vi "Parse String.vi"(8 "error in (no error)":errorcluster, 10 "Input String":string, 11 "ConfigManager.Text in":refnum<class "ConfigManager.Text.lvclass">) -> (0 "error out":errorcluster, 1 "Content":T1[](array[typedef]), 2 "Keys":string[](array[string]), 3 "ConfigManager.Text out":refnum<class "ConfigManager.Text.lvclass">, 5 "Section":string[](array[string]))   [LabVIEW 2013, in "CfgManager.Text.lvlib" / "ConfigManager.Text.lvclass"]
uses:
  ConfigManager.Text.lvclass
  Dictionary Payload -- cluster.ctl
  ConfigManager.Text.lvclass/ConfigManager.Text.ctl
  <vilib>/LabVIEW Open Source Project/Unicity/Delimiter/Delimiter.lvclass
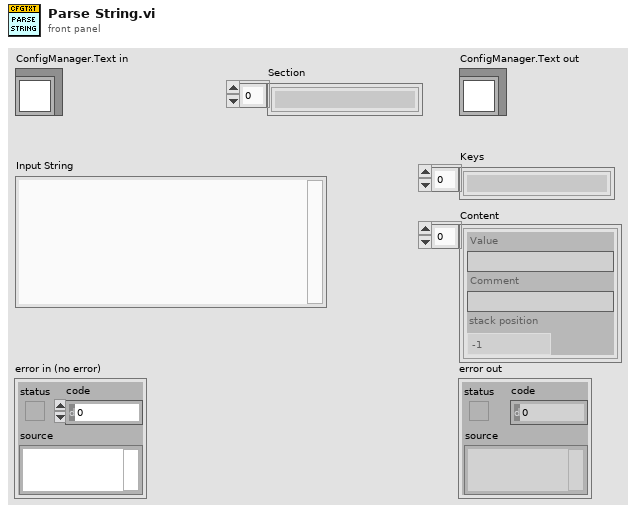
[diagram p1: front panel]
types:
  T1 = typedef "CfgManager.Text.lvlib/ConfigManager.Text.lvclass/Dictionary Payload -- cluster.ctl" = cluster{"Value":string, "Comment":string, "stack position":i32}
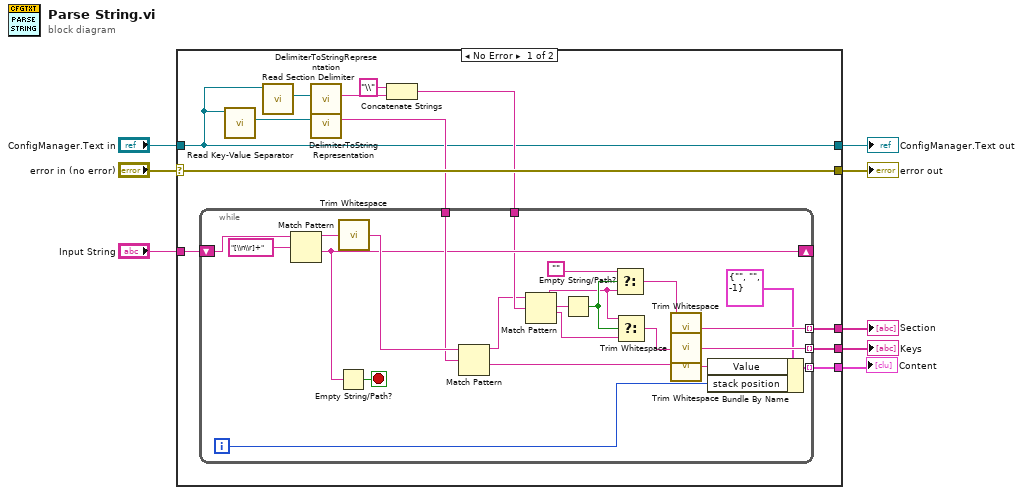
[diagram p0: block diagram]
diagram:
  n1 = case shown="No Error" "error in (no error)" {
    selector: "error in (no error)" -> [w20 w45]
    tunnel: [w20 w45] -> w7
    tunnel: [w10 w44] -> w5
    tunnel: "ConfigManager.Text in" -> [w10 w44]
    tunnel: "Input String" -> [w9 _]
    tunnel: [w19 _] -> w3
    tunnel: [w18 _] -> w1
    tunnel: [w16 _] -> w2
    frame No Error {
      n2 = call "Read Key-Value Separator.vi"("ConfigManager.Text in"=w10) -> ("Key Value Separator"=w11:refnum<class "Delimiter.lvclass">)  [unwired: 9 in, 1 out]
      n3 = call "Read Section Delimiter.vi"("ConfigManager.Text in"=w10) -> ("Section Delimiter"=w12:refnum<class "Delimiter.lvclass">)  [unwired: 9 in, 1 out]
      n4 = call <vilib>:"DelimiterToStringRepresentation.vi"("Delimiter"=w12) -> ("String representation"=w15:string)  [unwired: 10 in]
      n5 = call <vilib>:"DelimiterToStringRepresentation.vi"("Delimiter"=w11) -> ("String representation"=w17:string)  [unwired: 10 in]
      n6 = Concatenate Strings("\\" ("string"), w15) -> (w13:string)
      n7 = while {
        shift-right: [w35] -> _
        shift-left: w9 -> [w42]
        tunnel: [w38] -> w19 mode=indexing
        tunnel: w17 -> [w36]
        tunnel: [w22] -> w18 mode=indexing
        tunnel: [w30] -> w16 mode=indexing
        tunnel: w13 -> [w34]
        i -> [w21]
        stop <- w43 stop-if-true
        n8 = Match Pattern(string=w42, regular expression="[\\n\\r]+") -> (before substring=w41:string, after substring=w35:string)  [unwired: 1 in, 2 out]
        n9 = Empty String/Path?(string/path=w35) -> (empty?=w43:bool)
        n10 = call <vilib>:"Trim Whitespace.vi"("string"=w41) -> ("trimmed string"=w39:string)  [unwired: 1 in]
        n11 = Match Pattern(string=w39, regular expression=w36) -> (before substring=w26:string, after substring=w37:string)  [unwired: 1 in, 2 out]
        n12 = Match Pattern(string=w26, regular expression=w34) -> (before substring=w28:string, match substring=w33:string, after substring=w27:string)  [unwired: 1 in, 1 out]
        n13 = Empty String/Path?(string/path=w33) -> (empty?=w31:bool)
        n14 = Select(t="", s=w31, f=w28) -> (s? t:f=w29:string)
        n15 = Select(t=w28, s=w31, f=w27) -> (s? t:f=w25:string)
        n16 = call <vilib>:"Trim Whitespace.vi"("string"=w29) -> ("trimmed string"=w30:string)  [unwired: 1 in]
        n17 = call <vilib>:"Trim Whitespace.vi"("string"=w25) -> ("trimmed string"=w38:string)  [unwired: 1 in]
        n18 = call <vilib>:"Trim Whitespace.vi"("string"=w37) -> ("trimmed string"=w23:string)  [unwired: 1 in]
        n19 = Bundle By Name(cluster=T1 {"Value"="", "Comment"="", "stack position"=-1} ("Dictionary Payload"), "Value"=w23, "stack position"=w21) -> (w22:T1)
      }
    }
    frame Error {
    }
  }
  "error out" <- w7
  "ConfigManager.Text out" <- w5
  "Keys" <- w3
  "Content" <- w1
  "Section" <- w2
